vi "Test Generated Mock Class Creates When VIs.vi"(8 "error in (no error)":errorcluster, 11 "Test Case In":refnum<class "_Mock Class Generator Test.lvclass">) -> (0 "error out":errorcluster, 3 "Test Case Out":refnum<class "_Mock Class Generator Test.lvclass">)   [LabVIEW 2020, in "_Mock Class Generator Test.lvclass"]
uses:
  _Mock Class Generator Test.lvclass
  C:/Program Files (x86)/National Instruments/LabVIEW 2020/vi.lib/Astemes/LUnit/Test Case.lvclass
  <vilib>/Astemes/LUnit/Test Case.lvclass/Test Case.ctl
  <vilib>/Astemes/LUnit/Append Fail Result.vi
  <vilib>/Astemes/LUnit/Append Pass Result.vi
  <vilib>/Astemes/LUnit/Run In UI.vi
  <vilib>/Utility/error.llb/Clear Errors.vi
  _Mock Class Generator Test.lvclass/_Mock Class Generator Test.ctl
  source/Scripting/Mock Class Generator/Mock Class Generator.lvclass
  <vilib>/Astemes/LUnit/Test Case.lvclass
  C:/Program Files (x86)/National Instruments/LabVIEW 2020/vi.lib/Astemes/LUnit/LUnit Runnable.lvclass
  C:/git/astemes-lmock/tests/Mock Class Generator Test/_Mock Class Generator Test.lvclass
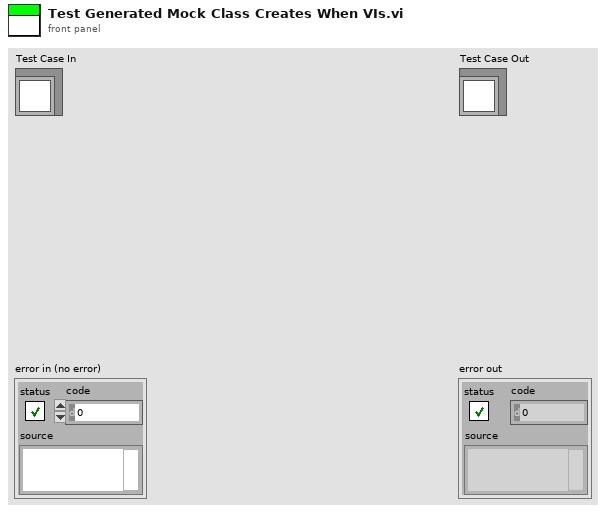
[diagram p1: front panel]
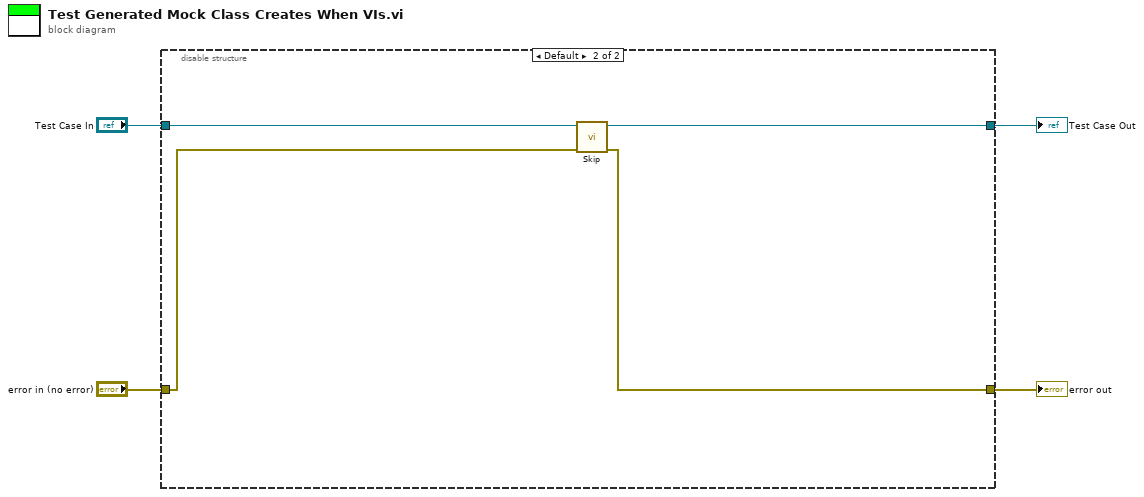
[diagram p0: block diagram]
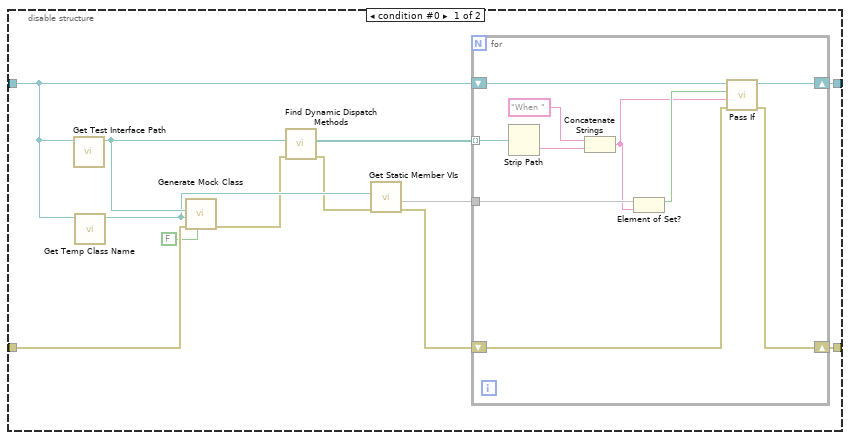
[diagram p2: hidden frame]
diagram:
  n1 = disable-structure shown="Default" {
    disable-tunnel: [w16 w27] -> w4
    disable-tunnel: [w15 w28] -> w3
    disable-tunnel: "Test Case In" -> [w14 w30]
    disable-tunnel: "error in (no error)" -> [w13 w29]
    frame condition #0 {
      n2 = call "Get Test Interface Path.vi"("Mock Class Generator Test in"=w14) -> ("Test Class Path"=w12:path)  [unwired: 10 in]
      n3 = call "Get Temp Class Name.vi"("Mock Class Generator Test in"=w14) -> ("Test Class Path"=w11:path)  [unwired: 10 in]
      n4 = call "Generate Mock Class.vi"("Add to lvproj?"=FALSE, "error in (no error)"=w13, "Destination Class Path"=w11, "Source Class Path"=w12) -> ("error out"=w9:errorcluster)  [unwired: 6 in, 1 out]
      n5 = call "Find Dynamic Dispatch Methods.vi"("error in (no error)"=w9, "Class Path"=w12) -> ("error out"=w10:errorcluster, "Dynamic Dispatch VIs"=w6:path[])  [unwired: 8 in]
      n6 = call "Get Static Member VIs.vi"("error in (no error)"=w10, "Test Class Path"=w11) -> ("error out"=w8:errorcluster, "VI Names"=w5:set{string})  [unwired: 7 in, 1 out]
      n7 = for {
        shift-right: [w26] -> w16
        shift-left: w14 -> [w24]
        shift-right: [w25] -> w15
        shift-left: w8 -> [w23]
        tunnel: w6 -> [w22] mode=indexing
        tunnel: w5 -> [w19]
        n8 = Strip Path(path=w22) -> (name=w21:string)  [unwired: 1 out]
        n9 = Concatenate Strings("When " ("string"), w21) -> (w17:string)
        n10 = Element of Set?(10:w17, 11:w19) -> (3:w18:bool)
        n11 = call <vilib>:"Pass If.vi"("error in (no error)"=w23, "Message"=w17, "Pass?"=w18, "LUnit Test Case In"=w24) -> ("error out"=w25:errorcluster, "LUnit Test Case Out"=w26:refnum<class "_Mock Class Generator Test.lvclass">)  [unwired: 6 in]
      }
    }
    frame condition #1 (active) {
      n12 = call <vilib>:"Skip.vi"("error in (no error)"=w29, "LUnit Test Case In"=w30) -> ("error out"=w28:errorcluster, "LUnit Test Case Out"=w27:refnum<class "_Mock Class Generator Test.lvclass">)  [unwired: 8 in]
    }
  }
  "error out" <- w3
  "Test Case Out" <- w4
